vi "Add Client Certificate Paths.vi"(10 "Client Connection Configuration In":T1) -> (2 "Client Connection Configuration Out":T1)   [LabVIEW 2014, in "OPC UA Client Tests.lvlib"]
doc: "Add Certificate paths to Client configuration"
uses:
  OPC UA Client Tests.lvlib
  module/configuration/Client Connection Configuration.ctl
  <vilib>/OPCUA/NI OPC UA Utility.lvlib
  module/configuration/OPC UA Client configuration.lvclass
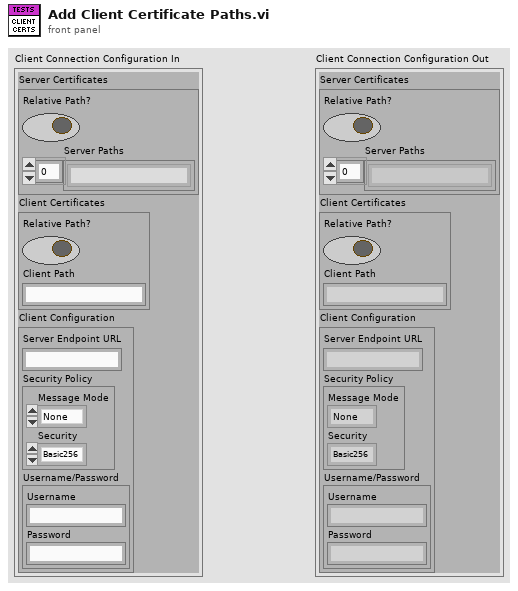
[diagram p1: front panel]
types:
  T1 = typedef "OPC UA Client configuration.lvclass/Client Connection Configuration.ctl" = cluster{"Server Certificates":cluster{"Relative Path?":bool, "Server Paths":string[]}, "Client Certificates":cluster{"Relative Path?":bool, "Client Path":string}, "Client Configuration":cluster{"Server Endpoint URL":string, "Security Policy":cluster{"Message Mode":enum16{"None", "Sign", "Sign and Encrypt"}, "Security":enum16{"Basic256", "Basic128Rsa15"}}, "Username/Password":cluster{"Username":string, "Password":string}}}
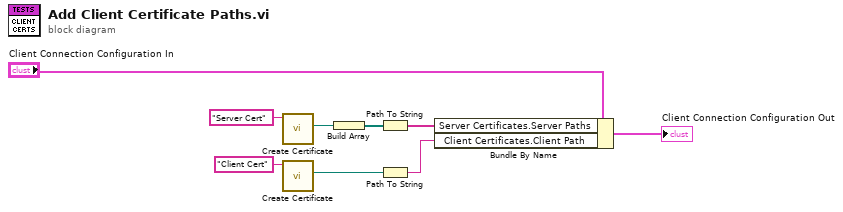
[diagram p0: block diagram]
diagram:
  n1 = call <vilib>:"Create Certificate.vi"("certificate name in"="Server Cert") -> ("certificate path"=w2:path)  [unwired: 7 in, 3 out]
  n2 = call <vilib>:"Create Certificate.vi"("certificate name in"="Client Cert") -> ("certificate path"=w1:path)  [unwired: 7 in, 3 out]
  n3 = Build Array(w2) -> (w9:path[])
  n4 = Path To String(path=w9) -> (string=w6:string[])
  n5 = Path To String(path=w1) -> (string=w5:string)
  n6 = Bundle By Name(cluster="Client Connection Configuration In", "Server Certificates.Server Paths"=w6, "Client Certificates.Client Path"=w5) -> (→"Client Connection Configuration Out":T1)
